vi "set NR HO Operation Band.vi"(8 "error in (no error)":errorcluster caption="에러 입력(에러 없음)", 9 "Selected CC Argements":T1, 10 "Operation Band":u32, 11 "Anritsu Call Box_Implement 입력":refnum<class "Anritsu Call Box_Implement.lvclass">) -> (0 "error out":errorcluster caption="에러 출력", 3 "Anritsu Call Box_Implement 출력":refnum<class "Anritsu Call Box_Implement.lvclass">)   [LabVIEW 2023, in "ANRITSU Call Box.lvlib" / "Anritsu Call Box_Implement.lvclass"]
uses:
  Anritsu Call Box_Implement.lvclass
  Anritsu Call Box_Implement.lvclass/Anritsu Call Box_Implement.ctl
  NR/NR.lvclass
  Type Definition/NR Selected CC Type Arguments.ctl
  ANRITSU Call Box.lvlib
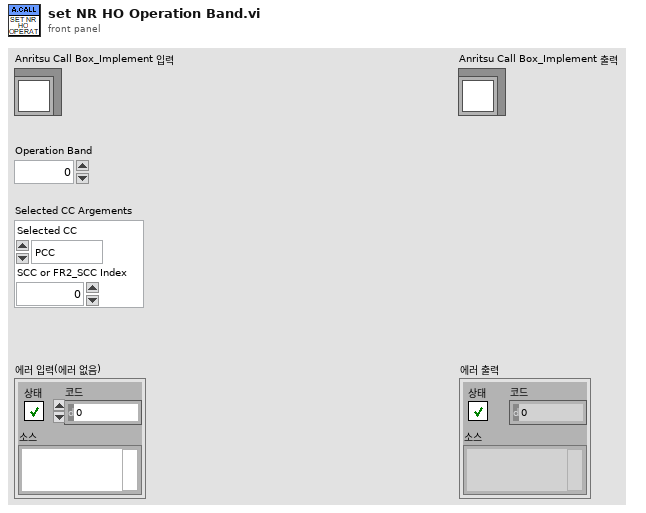
[diagram p1: front panel]
types:
  T1 = typedef "ANRITSU Call Box.lvlib/NR Selected CC Type Arguments.ctl" = cluster{"Selected CC":enum16{"PCC", "SCC", "FR2_PCC", "FR2_SCC"}, "SCC or FR2_SCC Index":u32}
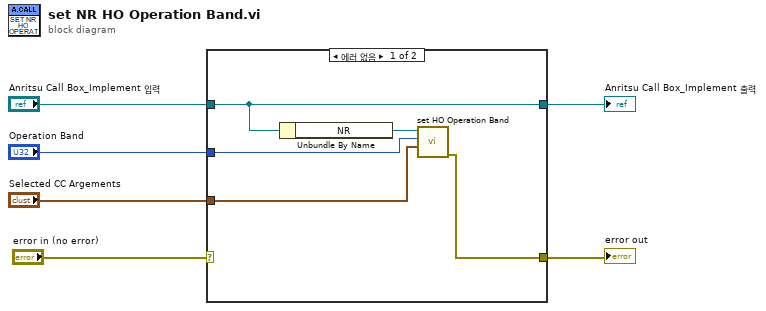
[diagram p0: block diagram]
diagram:
  n1 = case shown="에러 없음" "error in (no error)" {
    selector: "error in (no error)" -> [_ w13]
    tunnel: "Anritsu Call Box_Implement 입력" -> [w10 w12]
    tunnel: [w10 w12] -> w2
    tunnel: [w7 w13] -> w1
    tunnel: "Operation Band" -> [w9 _]
    tunnel: "Selected CC Argements" -> [w8 _]
    frame No Error {
      n2 = Unbundle By Name(w10) -> ("NR"=w11:refnum<class "NR.lvclass">)
      n3 = call "set HO Operation Band.vi"("Selected CC Argements"=w8, "Operation Band"=w9, "NR 입력"=w11) -> ("error out"=w7:errorcluster)  [unwired: 7 in, 1 out]
    }
    frame Error {
    }
  }
  "error out" <- w1
  "Anritsu Call Box_Implement 출력" <- w2
